vi "Delete Scale Wrapper.vi"(8 "error in":errorcluster, 10 "index":i32, 11 "Scaling configuration in":refnum<class "Scaling configuration.lvclass">) -> (0 "error out":errorcluster, 3 "Scaling configuration out":refnum<class "Scaling configuration.lvclass">)   [LabVIEW 2014, in "Scaling configuration.lvclass"]
uses:
  Scaling configuration.lvclass
  Scaling configuration.lvclass/Scaling configuration.ctl
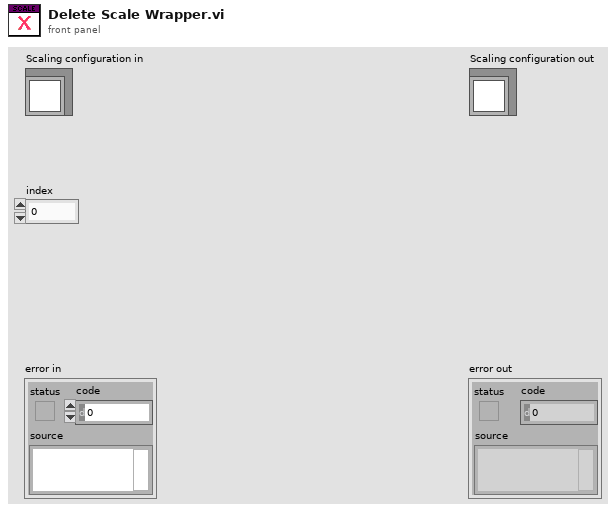
[diagram p1: front panel]
types:
  T1 = typedef "Scaling configuration.lvclass/scale data types.ctl" = enum16{"Double", "Single", "I64", "I32", "I16", "I8", "U64", "U32", "U16", "U8", "Boolean"}
  T2 = cluster{"mappings":cluster{"input channel":refnum<class "TBM channel.lvclass">, "output channel":refnum<class "TBM channel.lvclass">, "input data type":T1, "output data type":T1}[], "name":string}[]
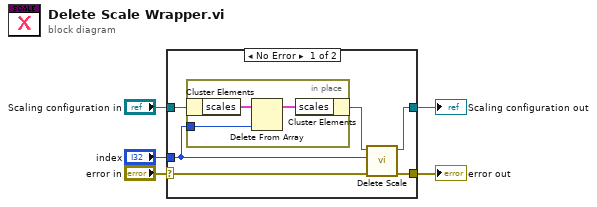
[diagram p0: block diagram]
diagram:
  n1 = case shown="No Error" "error in" {
    selector: "error in" -> [w8 w16]
    tunnel: [w7 w16] -> w4
    tunnel: [w6 w15] -> w2
    tunnel: "Scaling configuration in" -> [w11 w15]
    tunnel: "index" -> [w9 _]
    frame No Error {
      n2 = in-place {
        in-place-border: w9 -> [w13]
        n3 = in-place-cluster #1(w11) -> ("scales"=w14:T2)
        n4 = Delete From Array(array=w14, index=w13) -> (array with subset deleted=w12:T2)  [unwired: 1 in, 1 out]
        n5 = in-place-cluster #1("scales"=w12) -> (w10:refnum<class "Scaling configuration.lvclass">)
      }
      n6 = call-dynamic "Delete Scale.vi"("error in (no error)"=w8, "index"=w9, "Scaling configuration in"=w10) -> ("error out"=w7:errorcluster, "Scaling configuration out"=w6:refnum<class "Scaling configuration.lvclass">)  [unwired: 7 in]
    }
    frame Error {
    }
  }
  "error out" <- w4
  "Scaling configuration out" <- w2
